vi "Error Converter(ErrCheck).vi"(8 "error in (no error)":errorcluster, 10 "additional string":string="This error is returned by the shared library function.", 11 "status":i32) -> (0 "error out":errorcluster)   [LabVIEW 2023]
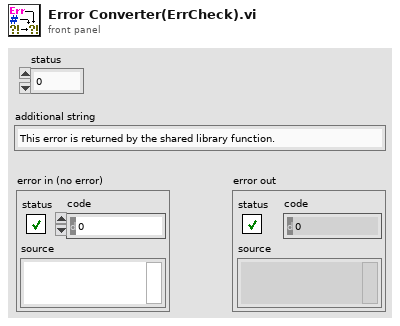
[diagram p1: front panel]
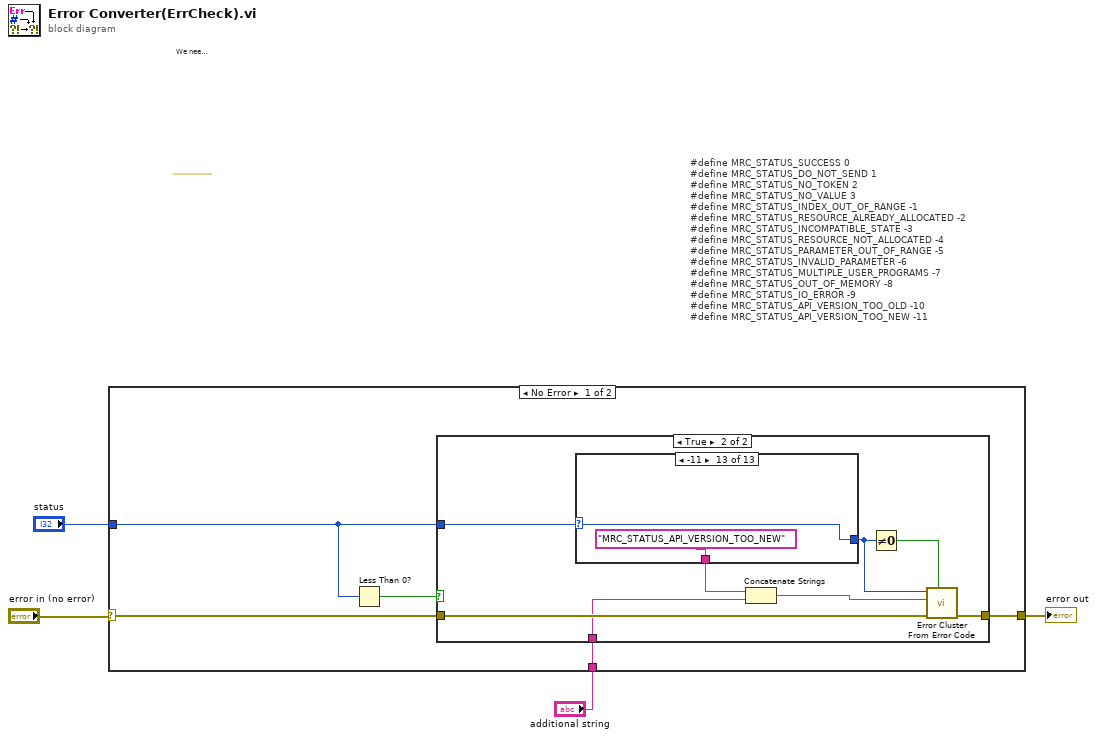
[diagram p0: block diagram]
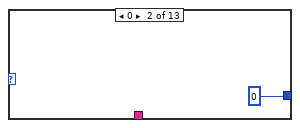
[diagram p4: hidden frame]
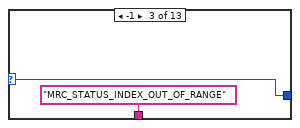
[diagram p5: hidden frame]
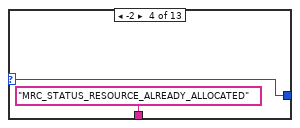
[diagram p6: hidden frame]
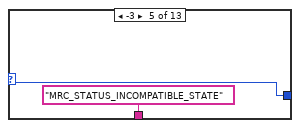
[diagram p7: hidden frame]
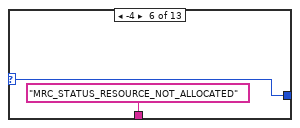
[diagram p8: hidden frame]
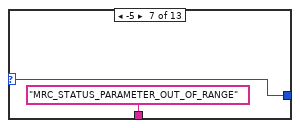
[diagram p9: hidden frame]
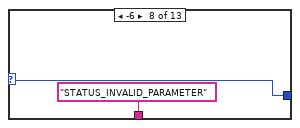
[diagram p10: hidden frame]
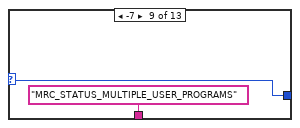
[diagram p11: hidden frame]
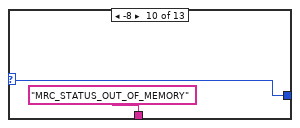
[diagram p12: hidden frame]
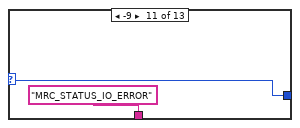
[diagram p13: hidden frame]
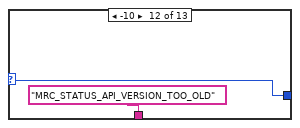
[diagram p14: hidden frame]
diagram:
  # "We need to map or wrap these status codes with LV clusters"
  # "#define MRC_STATUS_SUCCESS 0\n#define MRC_STATUS_DO_NOT_SEND 1\n#define MRC_STATUS_NO_TOKEN 2\n#define MRC_STATUS_NO_VALUE 3\n#define MRC_STATUS_INDEX_OUT_OF_RANGE -1\n#define MRC_STATUS_RESOURCE_ALREADY_ALLOCATED -2\n#define MRC_STATUS_INCOMPATIBLE_STATE -3\n#define MRC_STATUS_RESOURCE_NOT_ALLOCATED -4\n#define MRC_STATUS_PARAMETER_OUT_OF_RANGE -5\n#define MRC_STATUS_INVALID_PARAMETER -6\n#define MRC_STATUS_MULTIPLE_USER_PROGRAMS -7\n#define MRC_STATUS_OUT_OF_MEMORY -8\n#define MRC_STATUS_IO_ERROR -9\n#define MRC_STATUS_API_VERSION_TOO_OLD -10\n#define MRC_STATUS_API_VERSION_TOO_NEW -11"
  n1 = case shown="No Error" "error in (no error)" {
    selector: "error in (no error)" -> [w9 w43]
    tunnel: [w8 w43] -> w3
    tunnel: "status" -> [w6 _]
    tunnel: "additional string" -> [w7 _]
    frame No Error {
      n2 = Less Than 0?(x=w6) -> (x < 0?=w5:bool)
      n3 = case shown="True" w5 {
        tunnel: w9 -> [w10 w18]
        tunnel: [w10 w17] -> w8
        tunnel: w6 -> [_ w16]
        tunnel: w7 -> [_ w15]
        frame False {
        }
        frame True {
          n4 = case shown="-11" w16 {
            selector: w16 -> [w19 _ w22 w24 w26 w28 w30 w32 w34 w36 w38 w40 w42]
            tunnel: [w19 0 ("Error Code") w22 w24 w26 w28 w30 w32 w34 w36 w38 w40 w42] -> w14
            tunnel: [_ _ "MRC_STATUS_INDEX_OUT_OF_RANGE" "MRC_STATUS_RESOURCE_ALREADY_ALLOCATED" "MRC_STATUS_INCOMPATIBLE_STATE" "MRC_STATUS_RESOURCE_NOT_ALLOCATED" "MRC_STATUS_PARAMETER_OUT_OF_RANGE" "STATUS_INVALID_PARAMETER" "MRC_STATUS_MULTIPLE_USER_PROGRAMS" "MRC_STATUS_OUT_OF_MEMORY" "MRC_STATUS_IO_ERROR" "MRC_STATUS_API_VERSION_TOO_OLD" "MRC_STATUS_API_VERSION_TOO_NEW"] -> w11
            frame Default {
              # "what is this"
            }
            frame 0 {
              # "no error"
            }
            frame -1 {
              # "MRC_STATUS_INDEX_OUT_OF_RANGE"
            }
            frame -2 {
              # "MRC_STATUS_RESOURCE_ALREADY_ALLOCATED"
            }
            frame -3 {
              # "MRC_STATUS_INCOMPATIBLE_STATE"
            }
            frame -4 {
              # "MRC_STATUS_RESOURCE_NOT_ALLOCATED"
            }
            frame -5 {
              # "MRC_STATUS_PARAMETER_OUT_OF_RANGE"
            }
            frame -6 {
              # "MRC_STATUS_INVALID_PARAMETER"
            }
            frame -7 {
              # "MRC_STATUS_INVALID_PARAMETER"
            }
            frame -8 {
              # "MRC_STATUS_INVALID_PARAMETER"
            }
            frame -9 {
              # "MRC_STATUS_INVALID_PARAMETER"
            }
            frame -10 {
              # "MRC_STATUS_INVALID_PARAMETER"
            }
            frame -11 {
              # "MRC_STATUS_INVALID_PARAMETER"
            }
          }
          n5 = Concatenate Strings(w11, w15) -> (w12:string)
          n6 = Not Equal To 0?(x=w14) -> (x != 0?=w13:bool)
          n7 = call <vilib>:"Error Cluster From Error Code.vi"("show call chain? (False)"=w13, "error in (no error)"=w18, "error message (\"\")"=w12, "error code (0)"=w14) -> ("error out"=w17:errorcluster)  [unwired: 5 in]
        }
      }
    }
    frame Error {
    }
  }
  "error out" <- w3
